vi "Measurement Logic.vi"() -> ()   [LabVIEW 2021, in "Multi-Channel Output Voltage Accuracy_PMIC.lvlib"]
uses:
  Multi-Channel Output Voltage Accuracy_PMIC.lvlib
  Measurement Configuration.ctl
  Measurement Results.ctl
  <vilib>/Plug-In SDKs/Measurements/Measure Call Context/Measure Call Context.lvclass
  <instrlib>/niDCPower/nidcpower.llb/niDCPower Sense.ctl
  <instrlib>/niDCPower/nidcpower.llb/niDCPower Source Mode.ctl
  <instrlib>/niDCPower/nidcpower.llb/niDCPower Wait For Event - Event.ctl
  <instrlib>/niDCPower/nidcpower.llb/niDCPower Get Channel Name From String.vi
  <instrlib>/niDCPower/nidcpower.llb/niDCPower Configure Digital Edge Source Trigger.vi
  <instrlib>/niDCPower/nidcpower.llb/niDCPower Configure Digital Edge Measure Trigger.vi
panel:
  out "measure call context out":refnum<class "Measure Call Context.lvclass">
  in  "measure call context in":refnum<class "Measure Call Context.lvclass">
  out "measurement results":T1
  in  "measurement configuration":T2={"Mode of operation"=enum."Perform measurement", "DUT setup time"=1.0, "Aperture time"=0.005, "Measurement time"=1.0, "Source resource name"="", "Source sense"=1009, "Source voltage level"=6.0, "Source current limit"=10.0, "Load resource names"=[], "Load senses"=[], "Output channel alias"=[], "Load current levels"=[], "Load voltage limit ranges"=[], "Nominal Vout"=[]} {"Load senses" items=["Local"=1008, "Remote"=1009]; "Source sense" items=["Local"=1008, "Remote"=1009]; "Measurement time" format="%.3p"}
  out "error out":errorcluster
  in  "error in":errorcluster
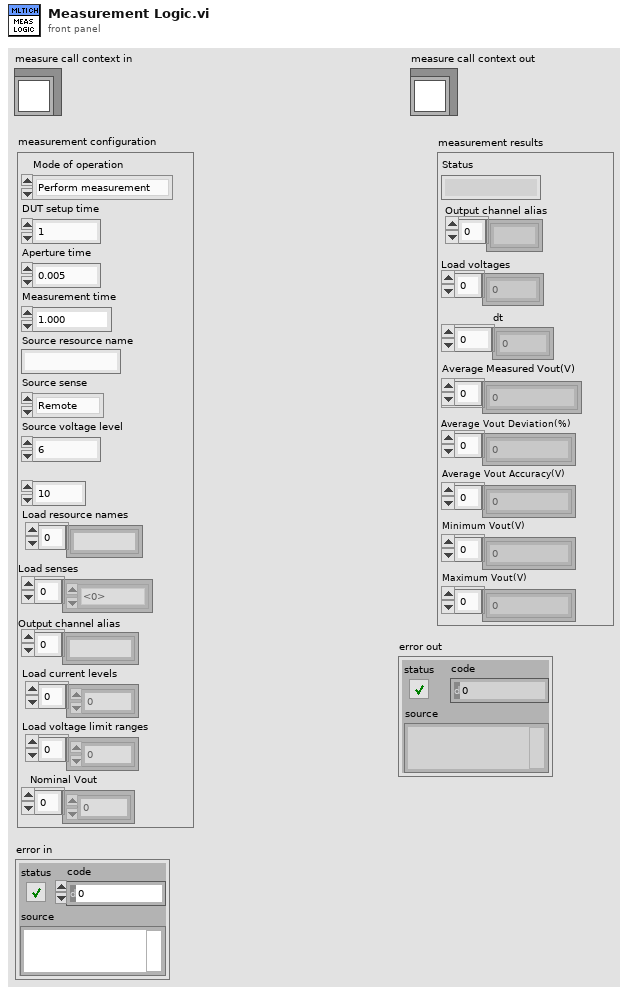
[diagram p1: front panel]
types:
  T1 = typedef "Multi-Channel Output Voltage Accuracy_PMIC.lvlib/Measurement Results.ctl" = cluster{"Status":string, "Output channel alias":string[], "Load voltages":dbl[], "dt":dbl[], "Average Measured Vout(V)":dbl[], "Average Vout Deviation(%)":dbl[], "Average Vout Accuracy(V)":dbl[], "Minimum Vout(V)":dbl[], "Maximum Vout(V)":dbl[]}
  T2 = typedef "Multi-Channel Output Voltage Accuracy_PMIC.lvlib/Measurement Configuration.ctl" = cluster{"Mode of operation":enum32{"Power on the DUT", "Perform measurement", "Power off the DUT"}, "DUT setup time":dbl, "Aperture time":dbl, "Measurement time":dbl, "Source resource name":string, "Source sense":i32, "Source voltage level":dbl, "Source current limit":dbl, "Load resource names":string[], "Load senses":i32[], "Output channel alias":string[], "Load current levels":dbl[], "Load voltage limit ranges":dbl[], "Nominal Vout":dbl[]}
  T3 = enum32{"Power on the DUT", "Perform measurement", "Power off the DUT"}
  T4 = typedef "niDCPower Wait For Event - Event.ctl" = i32
  T5 = typedef "niDCPower Source Mode.ctl" = i32
  T6 = typedef "niDCPower Sense.ctl" = i32
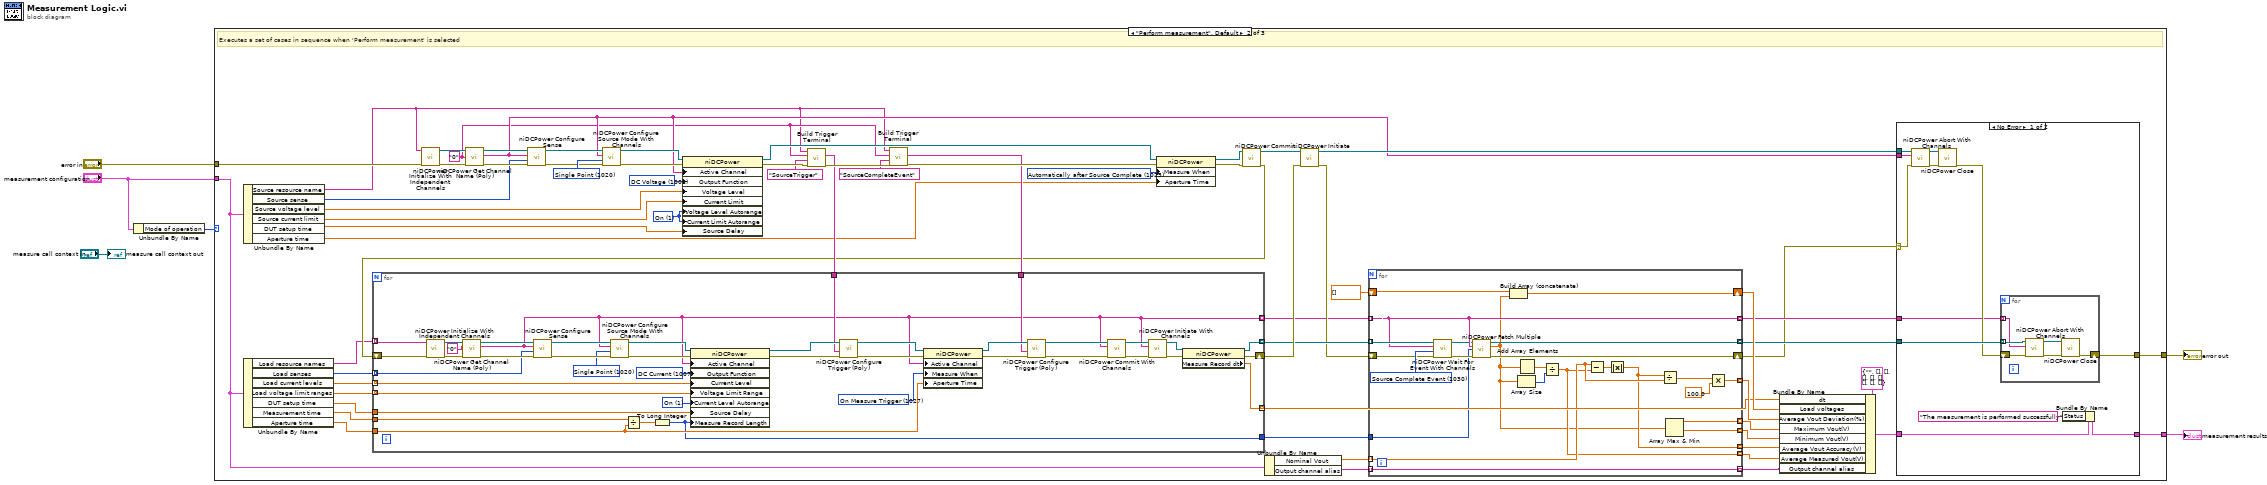
[diagram p0: block diagram]
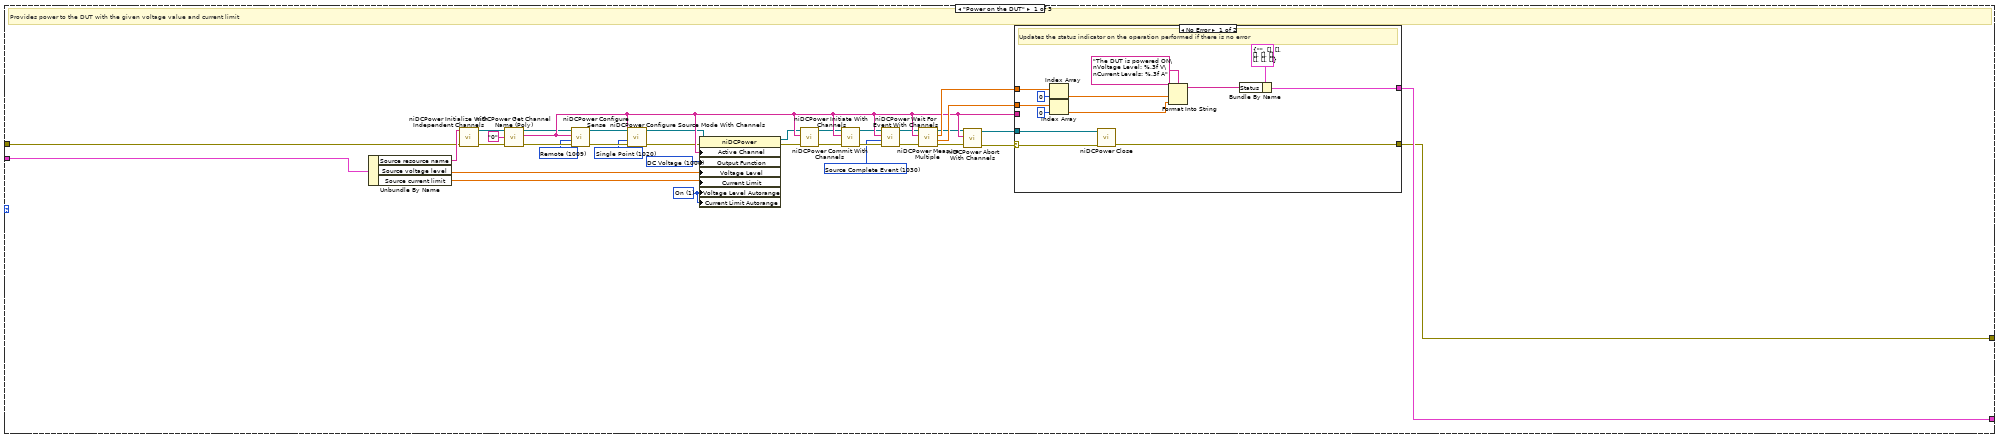
[diagram p2: hidden frame]
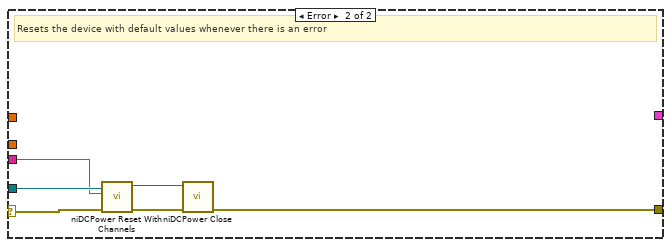
[diagram p3: hidden frame]
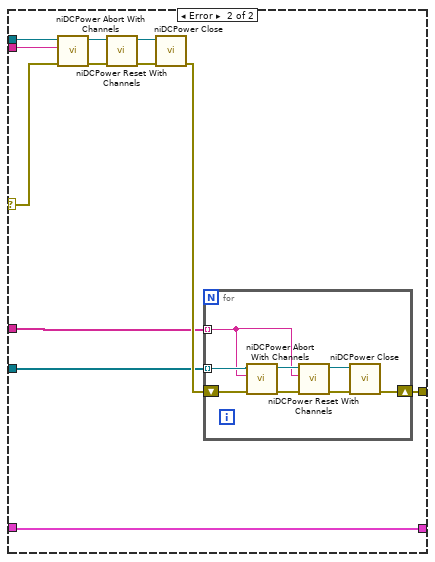
[diagram p4: hidden frame]
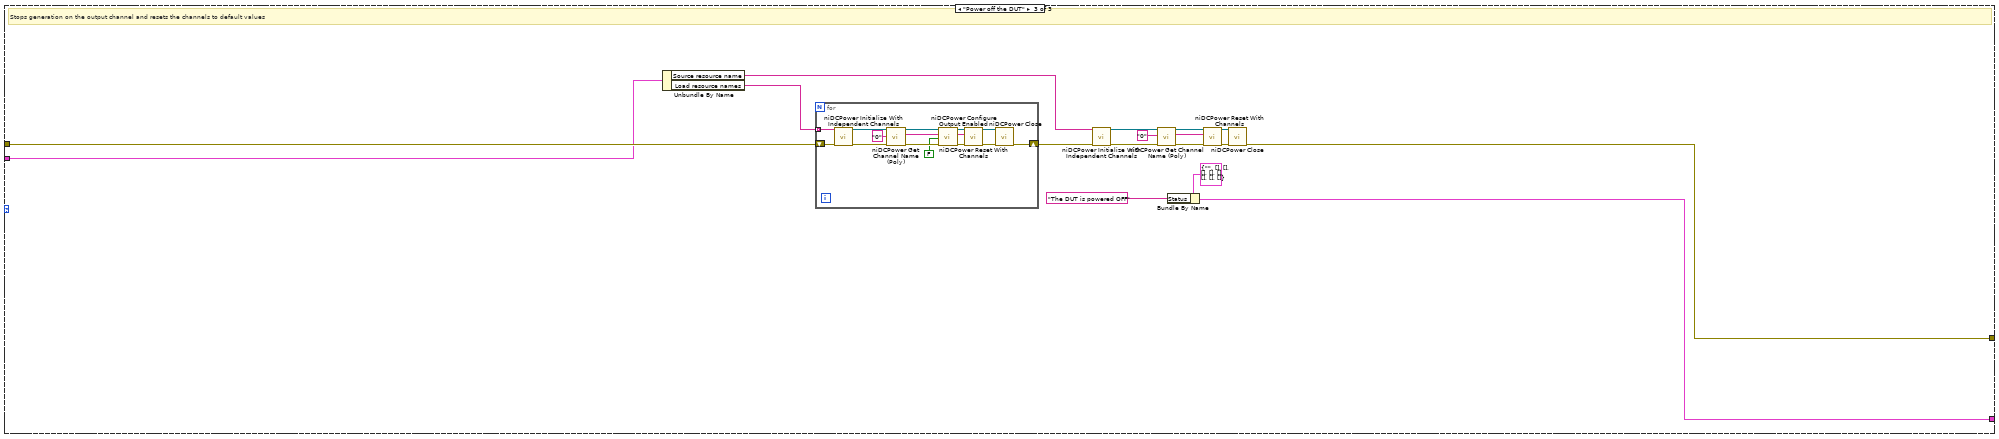
[diagram p5: hidden frame]
diagram:
  n1 = Unbundle By Name("measurement configuration") -> ("Mode of operation"=w4:T3)
  n2 = case shown="\"Perform measurement\", Default" w4 {
    tunnel: "measurement configuration" -> [w8 w94 w232]
    tunnel: "error in" -> [w10 w80 w233]
    tunnel: [w7 w79 w231] -> w2
    tunnel: [w9 w75 w229] -> w1
    frame "Power on the DUT" {
      w14 = 1 items=["Off", "On"] ("Source:DC Voltage:Voltage Level Autorange")
      w13 = T4 1030 items=["Source Complete Event"=1030, "Measure Complete Event"=1031, "Sequence Iteration Complete Event"=1032, "Sequence Engine Done Event"=1033, "Pulse Complete Event"=1051, "Ready For Pulse Trigger Event"=1052] ("event")
      w12 = T5 1020 items=["Single Point"=1020, "Sequence"=1021] ("source mode")
      w15 = 1006 items=["DC Voltage"=1006, "DC Current"=1007, "Pulse Voltage"=1049, "Pulse Current"=1050] ("Source:Output Function")
      w16 = T6 1009 items=["Local"=1008, "Remote"=1009] ("sense")
      # "Provides power to the DUT with the given voltage value and current limit"
      n3 = Unbundle By Name(w8) -> ("Source resource name"=w32:string, "Source voltage level"=w36:dbl, "Source current limit"=w31:dbl)
      n4 = call <instrlib>:"niDCPower Initialize With Independent Channels.vi"("error in (no error)"=w10, "resource name"=w32) -> ("error out"=w29:errorcluster, "instrument handle out"=w28:refnum<k15>)  [unwired: 8 in]
      n5 = call-poly <instrlib>:"niDCPower Get Channel Name (Poly).vi"("index"="0", "instrument handle"=w28) -> ("name"=w39:string, "instrument handle out"=w30:refnum<k15>)  [unwired: 7 in, 1 out]
      n6 = call <instrlib>:"niDCPower Configure Sense.vi"("error in (no error)"=w29, "sense"=w16, "channel name"=w39, "instrument handle"=w30) -> ("error out"=w22:errorcluster, "instrument handle out"=w24:refnum<k15>)  [unwired: 6 in]
      n7 = call <instrlib>:"niDCPower Configure Source Mode With Channels.vi"("error in (no error)"=w22, "source mode"=w12, "channel name"=w39, "instrument handle"=w24) -> ("error out"=w21:errorcluster, "instrument handle out"=w23:refnum<k15>)  [unwired: 6 in]
      n8 = property class="niDCPower"(reference=w23, error in=w21, "Active Channel"=w39, "Output Function"=w15, "Voltage Level"=w36, "Current Limit"=w31, "Voltage Level Autorange"=w14, "Current Limit Autorange"=w14) -> (reference out=w20:refnum<k15>, error out=w19:errorcluster)
      n9 = call <instrlib>:"niDCPower Commit With Channels.vi"("error in (no error)"=w19, "channel name"=w39, "instrument handle"=w20) -> ("error out"=w17:errorcluster, "instrument handle out"=w18:refnum<k15>)  [unwired: 7 in]
      n10 = call <instrlib>:"niDCPower Initiate With Channels.vi"("error in (no error)"=w17, "channel name"=w39, "instrument handle"=w18) -> ("error out"=w27:errorcluster, "instrument handle out"=w26:refnum<k15>)  [unwired: 7 in]
      n11 = call <instrlib>:"niDCPower Wait For Event With Channels.vi"("error in (no error)"=w27, "event"=w13, "channel name"=w39, "instrument handle"=w26) -> ("error out"=w34:errorcluster, "instrument handle out"=w25:refnum<k15>)  [unwired: 6 in]
      n12 = call <instrlib>:"niDCPower Measure Multiple.vi"("error in (no error)"=w34, "channel name"=w39, "instrument handle"=w25) -> ("error out"=w35:errorcluster, "current measurements"=w41:dbl[], "voltage measurements"=w40:dbl[], "instrument handle out"=w33:refnum<k15>)  [unwired: 5 in]
      n13 = call <instrlib>:"niDCPower Abort With Channels.vi"("error in (no error)"=w35, "channel name"=w39, "instrument handle"=w33) -> ("error out"=w37:errorcluster, "instrument handle out"=w38:refnum<k15>)  [unwired: 7 in]
      n14 = case shown="No Error" w37 {
        selector: w37 -> [w54 w58]
        tunnel: [w53 w57] -> w7
        tunnel: [w42 _] -> w9
        tunnel: w38 -> [w48 w56]
        tunnel: w39 -> [_ w55]
        tunnel: w40 -> [w47 _]
        tunnel: w41 -> [w46 _]
        frame No Error {
          # "Updates the status indicator on the operation performed if there is no error"
          n15 = Index Array(array=w47, index=0) -> (element=w45:dbl)
          n16 = Index Array(array=w46, index=0) -> (element=w44:dbl)
          n17 = call <instrlib>:"niDCPower Close.vi"("error in (no error)"=w54, "instrument handle"=w48) -> ("error out"=w53:errorcluster)  [unwired: 9 out]
          n18 = Format Into String(format string="The DUT is powered ON\nVoltage Level: %.3f V\nCurrent Levels: %.3f A" ("message"), w45, w44) -> (resulting string=w51:string)  [unwired: 2 in, 1 out]
          n19 = Bundle By Name(cluster=T1 {"Status"="", "Output channel alias"=[], "Load voltages"=[], "dt"=[], "Average Measured Vout(V)"=[], "Average Vout Deviation(%)"=[], "Average Vout Accuracy(V)"=[], "Minimum Vout(V)"=[], "Maximum Vout(V)"=[]} ("measurement results"), "Status"=w51) -> (w42:T1)
        }
        frame Error {
          # "Resets the device with default values whenever there is an error"
          n20 = call <instrlib>:"niDCPower Reset With Channels.vi"("error in (no error)"=w58, "channel name"=w55, "instrument handle"=w56) -> ("error out"=w60:errorcluster, "instrument handle out"=w59:refnum<k15>)  [unwired: 7 in]
          n21 = call <instrlib>:"niDCPower Close.vi"("error in (no error)"=w60, "instrument handle"=w59) -> ("error out"=w57:errorcluster)  [unwired: 9 out]
        }
      }
    }
    frame "Perform measurement", Default {
      w115 = 1025 items=["Automatically after Source Complete"=1025, "On Demand"=1026, "On Measure Trigger"=1027] ("Measurement:Advanced:Measure When")
      w70 = "0" ("index")
      w119 = 1 items=["Off", "On"] ("Source:DC Voltage:Voltage Level Autorange")
      w125 = T5 1020 items=["Single Point"=1020, "Sequence"=1021] ("source mode")
      w121 = 1006 items=["DC Voltage"=1006, "DC Current"=1007, "Pulse Voltage"=1049, "Pulse Current"=1050] ("Source:Output Function")
      # "Executes a set of cases in sequence when 'Perform measurement' is selected"
      n22 = Unbundle By Name(w94) -> ("Source resource name"=w62:string, "Source sense"=w61:i32, "Source voltage level"=w111:dbl, "Source current limit"=w110:dbl, "DUT setup time"=w109:dbl, "Aperture time"=w81:dbl)
      n23 = Unbundle By Name(w94) -> ("Load resource names"=w64:string[], "Load senses"=w63:i32[], "Load current levels"=w103:dbl[], "Load voltage limit ranges"=w102:dbl[], "DUT setup time"=w101:dbl, "Measurement time"=w95:dbl, "Aperture time"=w96:dbl)
      n24 = call <instrlib>:"niDCPower Initialize With Independent Channels.vi"("error in (no error)"=w80, "resource name"=w62) -> ("error out"=w69:errorcluster, "instrument handle out"=w120:refnum<k15>)  [unwired: 8 in]
      n25 = call-poly <instrlib>:"niDCPower Get Channel Name (Poly).vi"("error in (no error)"=w69, "index"=w70, "instrument handle"=w120) -> ("error out"=w68:errorcluster, "name"=w71:string, "instrument handle out"=w118:refnum<k15>)  [unwired: 6 in]
      n26 = call <instrlib>:"niDCPower Configure Sense.vi"("error in (no error)"=w68, "sense"=w61, "channel name"=w71, "instrument handle"=w118) -> ("error out"=w123:errorcluster, "instrument handle out"=w122:refnum<k15>)  [unwired: 6 in]
      n27 = call <instrlib>:"niDCPower Configure Source Mode With Channels.vi"("error in (no error)"=w123, "source mode"=w125, "channel name"=w71, "instrument handle"=w122) -> ("error out"=w124:errorcluster, "instrument handle out"=w108:refnum<k15>)  [unwired: 6 in]
      n28 = property class="niDCPower"(reference=w108, error in=w124, "Active Channel"=w71, "Output Function"=w121, "Voltage Level"=w111, "Current Limit"=w110, "Voltage Level Autorange"=w119, "Current Limit Autorange"=w119, "Source Delay"=w109) -> (reference out=w107:refnum<k15>, error out=w114:errorcluster)
      n29 = call "Build Trigger Terminal.vi"("error in (no error)"=w114, "Trigger/Event Name"="SourceTrigger", "Channel Name"=w70, "Resource Name"=w62) -> ("error out"=w113:errorcluster, "Terminal Name"=w106:string)  [unwired: 6 in]
      n30 = call "Build Trigger Terminal.vi"("error in (no error)"=w113, "Trigger/Event Name"="SourceCompleteEvent", "Channel Name"=w70, "Resource Name"=w62) -> ("error out"=w112:errorcluster, "Terminal Name"=w105:string)  [unwired: 6 in]
      n31 = property class="niDCPower"(reference=w107, error in=w112, "Measure When"=w115, "Aperture Time"=w81) -> (reference out=w117:refnum<k15>, error out=w116:errorcluster)
      n32 = call <instrlib>:"niDCPower Commit.vi"("error in (no error)"=w116, "instrument handle"=w117) -> ("error out"=w104:errorcluster, "instrument handle out"=w100:refnum<k15>)  [unwired: 8 out]
      n33 = for {
        tunnel: w96 -> [w198]
        tunnel: [w193] -> w98 mode=indexing
        tunnel: w106 -> [w206]
        tunnel: w105 -> [w205]
        tunnel: w101 -> [w201]
        shift-right: [w195] -> w99
        shift-left: w104 -> [w207]
        tunnel: w64 -> [w204] mode=indexing
        tunnel: w103 -> [w203] mode=indexing
        tunnel: w102 -> [w202] mode=indexing
        tunnel: w95 -> [w200]
        tunnel: [w197] -> w78
        tunnel: [w191] -> w83 mode=indexing
        tunnel: [w192] -> w65 mode=indexing
        tunnel: w63 -> [w188] mode=indexing
        w212 = 1027 items=["Automatically after Source Complete"=1025, "On Demand"=1026, "On Measure Trigger"=1027] ("Measurement:Advanced:Measure When")
        w217 = 1 items=["Off", "On"] ("Source:DC Current:Current Level Autorange")
        w218 = 1007 items=["DC Voltage"=1006, "DC Current"=1007, "Pulse Voltage"=1049, "Pulse Current"=1050] ("Source:Output Function")
        w221 = T5 1020 items=["Single Point"=1020, "Sequence"=1021] ("source mode")
        n34 = call <instrlib>:"niDCPower Initialize With Independent Channels.vi"("error in (no error)"=w207, "resource name"=w204) -> ("error out"=w190:errorcluster, "instrument handle out"=w226:refnum<k15>)  [unwired: 8 in]
        n35 = call-poly <instrlib>:"niDCPower Get Channel Name (Poly).vi"("error in (no error)"=w190, "index"="0", "instrument handle"=w226) -> ("error out"=w189:errorcluster, "name"=w191:string, "instrument handle out"=w227:refnum<k15>)  [unwired: 6 in]
        n36 = call <instrlib>:"niDCPower Configure Sense.vi"("error in (no error)"=w189, "sense"=w188, "channel name"=w191, "instrument handle"=w227) -> ("error out"=w223:errorcluster, "instrument handle out"=w225:refnum<k15>)  [unwired: 6 in]
        n37 = call <instrlib>:"niDCPower Configure Source Mode With Channels.vi"("error in (no error)"=w223, "source mode"=w221, "channel name"=w191, "instrument handle"=w225) -> ("error out"=w222:errorcluster, "instrument handle out"=w224:refnum<k15>)  [unwired: 6 in]
        n38 = Divide(x=w200, y=w198) -> (x/y=w199:dbl)
        n39 = To Long Integer(number=w199) -> (32bit integer=w197:i32)
        n40 = property class="niDCPower"(reference=w224, error in=w222, "Active Channel"=w191, "Output Function"=w218, "Current Level"=w203, "Voltage Limit Range"=w202, "Current Level Autorange"=w217, "Source Delay"=w201, "Measure Record Length"=w197) -> (reference out=w208:refnum<k15>, error out=w211:errorcluster)
        n41 = call-poly <instrlib>:"niDCPower Configure Trigger (Poly).vi"("error in (no error)"=w211, "input terminal"=w206, "instrument handle"=w208) -> ("error out"=w215:errorcluster, "instrument handle out"=w216:refnum<k15>)  [unwired: 1 in, 6 out]
        n42 = property class="niDCPower"(reference=w216, error in=w215, "Active Channel"=w191, "Measure When"=w212, "Aperture Time"=w198) -> (reference out=w213:refnum<k15>, error out=w214:errorcluster)
        n43 = call-poly <instrlib>:"niDCPower Configure Trigger (Poly).vi"("error in (no error)"=w214, "input terminal"=w205, "instrument handle"=w213) -> ("error out"=w210:errorcluster, "instrument handle out"=w209:refnum<k15>)  [unwired: 1 in, 6 out]
        n44 = call <instrlib>:"niDCPower Commit With Channels.vi"("error in (no error)"=w210, "channel name"=w191, "instrument handle"=w209) -> ("error out"=w220:errorcluster, "instrument handle out"=w219:refnum<k15>)  [unwired: 7 in]
        n45 = call <instrlib>:"niDCPower Initiate With Channels.vi"("error in (no error)"=w220, "channel name"=w191, "instrument handle"=w219) -> ("error out"=w196:errorcluster, "instrument handle out"=w194:refnum<k15>)  [unwired: 7 in]
        n46 = property class="niDCPower"(reference=w194, error in=w196) -> (reference out=w193:refnum<k15>, error out=w195:errorcluster, "Measure Record dt"=w192:dbl)
      }
      n47 = Unbundle By Name(w94) -> ("Nominal Vout"=w93:dbl[], "Output channel alias"=w92:string[])
      n48 = call <instrlib>:"niDCPower Initiate.vi"("error in (no error)"=w99, "instrument handle"=w100) -> ("error out"=w97:errorcluster, "instrument handle out"=w84:refnum<k15>)  [unwired: 8 out]
      n49 = for {
        shift-right: [w169] -> w74
        shift-left: w97 -> [w186]
        tunnel: [w171] -> w85 mode=indexing
        tunnel: w98 -> [w185] mode=indexing
        tunnel: w93 -> [w179] mode=indexing
        tunnel: [w167] -> w77 mode=indexing
        tunnel: [w178] -> w88 mode=indexing
        tunnel: [w177] -> w89 mode=indexing
        tunnel: [w176] -> w90 mode=indexing
        tunnel: w92 -> [w176] mode=indexing
        shift-right: [w174] -> w86
        shift-left: dbl[] [] -> [w175]
        tunnel: w83 -> [w173] mode=indexing
        tunnel: [w173] -> w82 mode=indexing
        tunnel: w78 -> [w168]
        tunnel: [w165] -> w67 mode=indexing
        tunnel: [w164] -> w66 mode=indexing
        w187 = T4 1030 items=["Source Complete Event"=1030, "Measure Complete Event"=1031, "Sequence Iteration Complete Event"=1032, "Sequence Engine Done Event"=1033, "Pulse Complete Event"=1051, "Ready For Pulse Trigger Event"=1052] ("event")
        n50 = call <instrlib>:"niDCPower Wait For Event With Channels.vi"("error in (no error)"=w186, "event"=w187, "channel name"=w173, "instrument handle"=w185) -> ("error out"=w170:errorcluster, "instrument handle out"=w172:refnum<k15>)  [unwired: 6 in]
        n51 = call <instrlib>:"niDCPower Fetch Multiple.vi"("instrument handle"=w172, "channel name"=w173, "count (1)"=w168, "error in (no error)"=w170) -> ("instrument handle out"=w171:refnum<k15>, "voltage measurements"=w166:dbl[], "error out"=w169:errorcluster)  [unwired: 6 in, 3 out]
        n52 = Build Array (concatenate)(w175, w166) -> (w174:dbl[])
        n53 = Add Array Elements(numeric array=w166) -> (sum=w181:dbl)
        n54 = Array Size(array=w166) -> (size(s)=w180:i32)
        n55 = Divide(x=w181, y=w180) -> (x/y=w177:dbl)
        n56 = Subtract(x=w179, y=w177) -> (x-y=w182:dbl)
        n57 = Absolute Value(x=w182) -> (abs(x)=w167:dbl)
        n58 = Divide(x=w167, y=w179) -> (x/y=w184:dbl)
        n59 = Array Max & Min(array=w166) -> (max value=w165:dbl, min value=w164:dbl)  [unwired: 2 out]
        n60 = Multiply(x=w184, y=100.0) -> (x*y=w178:dbl)
      }
      n61 = Bundle By Name(cluster=T1 {"Status"="", "Output channel alias"=[], "Load voltages"=[], "dt"=[], "Average Measured Vout(V)"=[], "Average Vout Deviation(%)"=[], "Average Vout Accuracy(V)"=[], "Minimum Vout(V)"=[], "Maximum Vout(V)"=[]} ("measurement results"), "dt"=w65, "Load voltages"=w86, "Average Vout Deviation(%)"=w88, "Maximum Vout(V)"=w67, "Minimum Vout(V)"=w66, "Average Vout Accuracy(V)"=w77, "Average Measured Vout(V)"=w89, "Output channel alias"=w90) -> (w76:T1)
      n62 = case shown="No Error" w74 {
        selector: w74 -> [w126 w146]
        tunnel: w85 -> [w137 w154]
        tunnel: w84 -> [w133 w152]
        tunnel: w82 -> [w132 w153]
        tunnel: [w131 w145] -> w79
        tunnel: w71 -> [w130 w151]
        tunnel: w76 -> [w128 w144]
        tunnel: [w129 w144] -> w75
        frame No Error {
          n63 = call <instrlib>:"niDCPower Abort With Channels.vi"("error in (no error)"=w126, "channel name"=w130, "instrument handle"=w133) -> ("error out"=w136:errorcluster, "instrument handle out"=w135:refnum<k15>)  [unwired: 7 in]
          n64 = call <instrlib>:"niDCPower Close.vi"("error in (no error)"=w136, "instrument handle"=w135) -> ("error out"=w134:errorcluster)  [unwired: 9 out]
          n65 = for {
            shift-right: [w142] -> w131
            shift-left: w134 -> [w143]
            tunnel: w137 -> [w139] mode=indexing
            tunnel: w132 -> [w138] mode=indexing
            n66 = call <instrlib>:"niDCPower Abort With Channels.vi"("error in (no error)"=w143, "channel name"=w138, "instrument handle"=w139) -> ("error out"=w141:errorcluster, "instrument handle out"=w140:refnum<k15>)  [unwired: 7 in]
            n67 = call <instrlib>:"niDCPower Close.vi"("error in (no error)"=w141, "instrument handle"=w140) -> ("error out"=w142:errorcluster)  [unwired: 9 out]
          }
          n68 = Bundle By Name(cluster=w128, "Status"="The measurement is performed successfully" ("message")) -> (w129:T1)
        }
        frame Error {
          n69 = call <instrlib>:"niDCPower Abort With Channels.vi"("error in (no error)"=w146, "channel name"=w151, "instrument handle"=w152) -> ("error out"=w148:errorcluster, "instrument handle out"=w150:refnum<k15>)  [unwired: 7 in]
          n70 = call <instrlib>:"niDCPower Reset With Channels.vi"("error in (no error)"=w148, "instrument handle"=w150) -> ("error out"=w147:errorcluster, "instrument handle out"=w149:refnum<k15>)  [unwired: 8 in]
          n71 = call <instrlib>:"niDCPower Close.vi"("error in (no error)"=w147, "instrument handle"=w149) -> ("error out"=w155:errorcluster)  [unwired: 9 out]
          n72 = for {
            shift-right: [w162] -> w145
            shift-left: w155 -> [w163]
            tunnel: w154 -> [w161] mode=indexing
            tunnel: w153 -> [w156] mode=indexing
            n73 = call <instrlib>:"niDCPower Abort With Channels.vi"("error in (no error)"=w163, "channel name"=w156, "instrument handle"=w161) -> ("error out"=w160:errorcluster, "instrument handle out"=w158:refnum<k15>)  [unwired: 7 in]
            n74 = call <instrlib>:"niDCPower Reset With Channels.vi"("error in (no error)"=w160, "channel name"=w156, "instrument handle"=w158) -> ("error out"=w159:errorcluster, "instrument handle out"=w157:refnum<k15>)  [unwired: 7 in]
            n75 = call <instrlib>:"niDCPower Close.vi"("error in (no error)"=w159, "instrument handle"=w157) -> ("error out"=w162:errorcluster)  [unwired: 9 out]
          }
        }
      }
    }
    frame "Power off the DUT" {
      # "Stops generation on the output channel and resets the channels to default values"
      n76 = Unbundle By Name(w232) -> ("Source resource name"=w244:string, "Load resource names"=w242:string[])
      n77 = for {
        tunnel: w242 -> [w258] mode=indexing
        shift-right: [w256] -> w239
        shift-left: w233 -> [w246]
        n78 = call <instrlib>:"niDCPower Initialize With Independent Channels.vi"("error in (no error)"=w246, "resource name"=w258) -> ("error out"=w257:errorcluster, "instrument handle out"=w259:refnum<k15>)  [unwired: 8 in]
        n79 = call-poly <instrlib>:"niDCPower Get Channel Name (Poly).vi"("error in (no error)"=w257, "index"="0", "instrument handle"=w259) -> ("error out"=w253:errorcluster, "name"=w255:string, "instrument handle out"=w254:refnum<k15>)  [unwired: 6 in]
        n80 = call <instrlib>:"niDCPower Configure Output Enabled.vi"("error in (no error)"=w253, "output enabled"=FALSE, "channel name"=w255, "instrument handle"=w254) -> ("error out"=w249:errorcluster, "instrument handle out"=w250:refnum<k15>)  [unwired: 6 in]
        n81 = call <instrlib>:"niDCPower Reset With Channels.vi"("error in (no error)"=w249, "channel name"=w255, "instrument handle"=w250) -> ("error out"=w252:errorcluster, "instrument handle out"=w251:refnum<k15>)  [unwired: 7 in]
        n82 = call <instrlib>:"niDCPower Close.vi"("error in (no error)"=w252, "instrument handle"=w251) -> ("error out"=w256:errorcluster)  [unwired: 9 out]
      }
      n83 = call <instrlib>:"niDCPower Initialize With Independent Channels.vi"("error in (no error)"=w239, "resource name"=w244) -> ("error out"=w243:errorcluster, "instrument handle out"=w245:refnum<k15>)  [unwired: 8 in]
      n84 = call-poly <instrlib>:"niDCPower Get Channel Name (Poly).vi"("error in (no error)"=w243, "index"="0", "instrument handle"=w245) -> ("error out"=w240:errorcluster, "name"=w241:string, "instrument handle out"=w238:refnum<k15>)  [unwired: 6 in]
      n85 = Bundle By Name(cluster=T1 {"Status"="", "Output channel alias"=[], "Load voltages"=[], "dt"=[], "Average Measured Vout(V)"=[], "Average Vout Deviation(%)"=[], "Average Vout Accuracy(V)"=[], "Minimum Vout(V)"=[], "Maximum Vout(V)"=[]} ("measurement results"), "Status"="The DUT is powered OFF" ("Measurement Results.Status")) -> (w229:T1)
      n86 = call <instrlib>:"niDCPower Reset With Channels.vi"("error in (no error)"=w240, "channel name"=w241, "instrument handle"=w238) -> ("error out"=w236:errorcluster, "instrument handle out"=w237:refnum<k15>)  [unwired: 7 in]
      n87 = call <instrlib>:"niDCPower Close.vi"("error in (no error)"=w236, "instrument handle"=w237) -> ("error out"=w231:errorcluster)  [unwired: 9 out]
    }
  }
  "error out" <- w2
  "measurement results" <- w1
  "measure call context out" <- "measure call context in"
